vi "LoadCFG.vi"(8 "error in (no error)":errorcluster, 11 "object in":refnum<class "AIO-Configuration.lvclass">) -> (0 "error out":errorcluster, 2 "Success?":bool, 3 "object out":refnum<class "AIO-Configuration.lvclass">)   [LabVIEW 2021, in "DAQmx.lvlib" / "AIO-Configuration.lvclass"]
doc: "Loads Configuration"
uses:
  AIO-Configuration.lvclass
  C:/Users/averna/Documents/LV Gym DEMO/Factory Pattern/Channels/Dependencies/Channel.lvlibp/Channel/Configuration_class/Configuration.lvclass
  tdef/Data.ctl
  AIO-Configuration.lvclass/AIO-Configuration.ctl
  Dependencies/Channel.lvlibp/Channel/Configuration_class/properties/ReadConfigurationFile.vi
  <vilib>/Utility/config.llb/Read Key (String).vi
  <vilib>/Utility/config.llb/Read Key (Double).vi
  Dependencies/AIO-Channel.lvlibp/AIO-Configuration_class/AIO-Configuration.lvclass
  <vilib>/Utility/config.llb/NI_LVConfig.lvlib
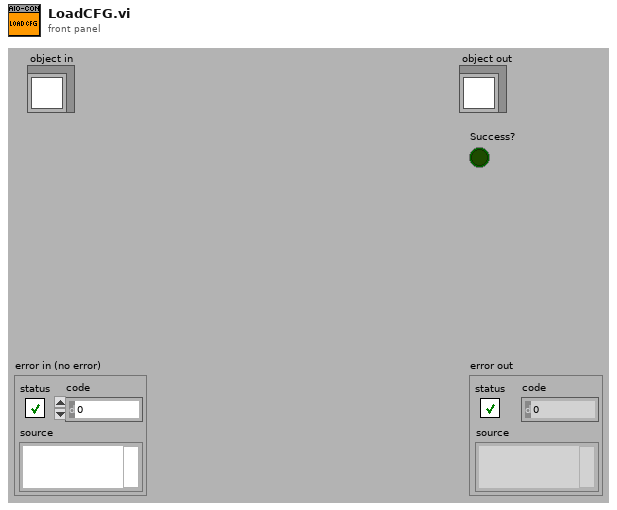
[diagram p1: front panel]
types:
  T1 = typedef "DAQmx.lvlib/AIO-Configuration.lvclass/Data.ctl" = cluster{"DAQ_Line":string, "maximum value":dbl, "minimum value":dbl, "input terminal configuration":i32, "custom scale name":string}
  T2 = typedef "NI_LVConfig.lvlib/Config Data RefNum.ctl" = refnum<k1>
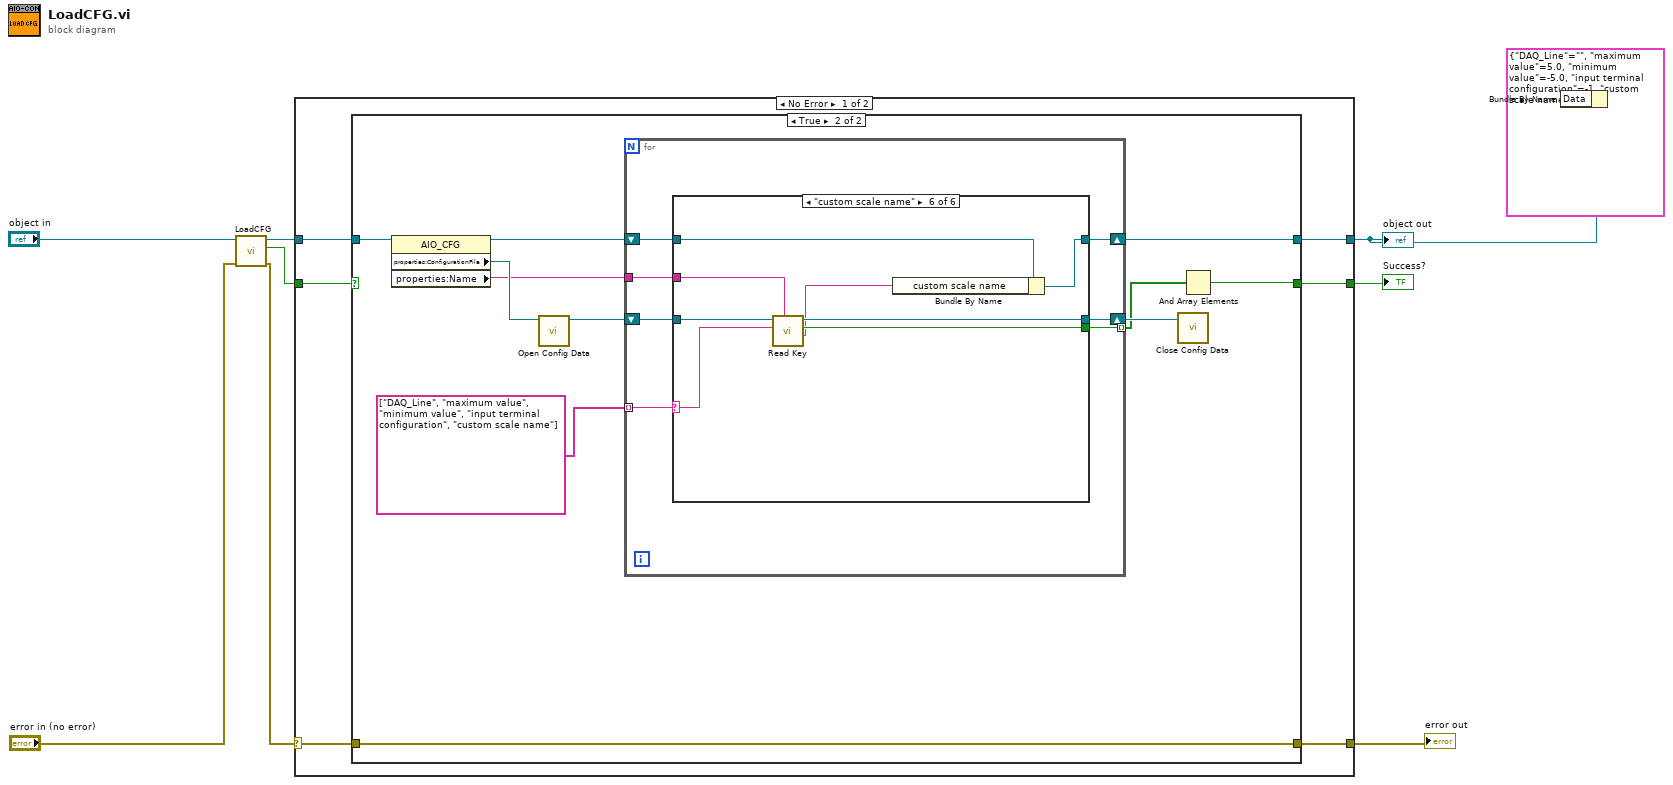
[diagram p0: block diagram]
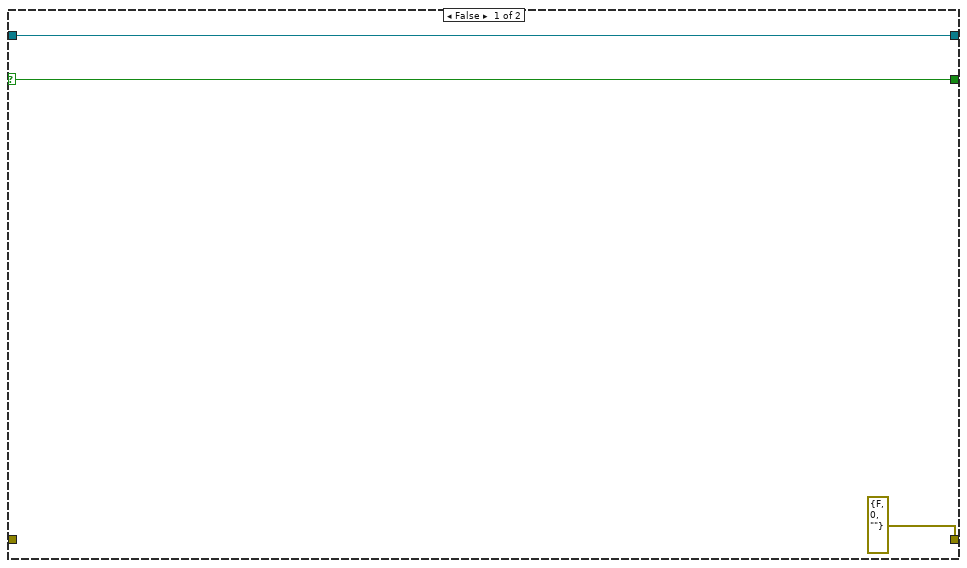
[diagram p2: hidden frame]
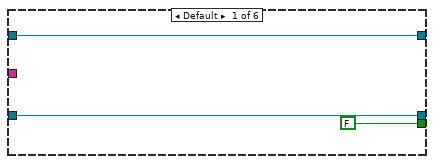
[diagram p3: hidden frame]
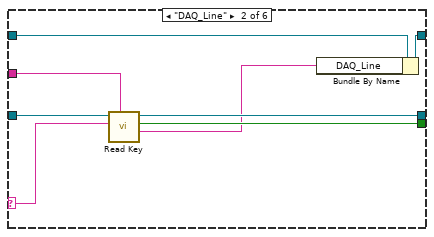
[diagram p4: hidden frame]
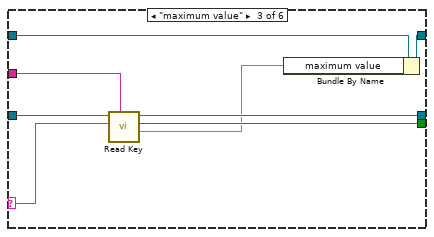
[diagram p5: hidden frame]
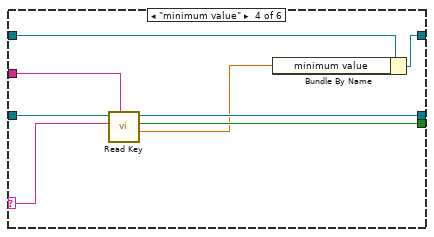
[diagram p6: hidden frame]
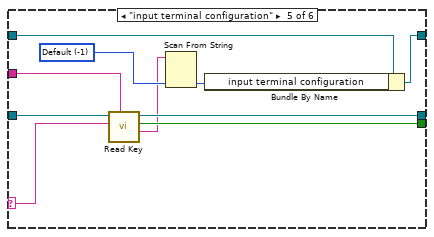
[diagram p7: hidden frame]
diagram:
  n1 = call-parent "LoadCFG.vi"("error in (no error)"="error in (no error)", "object in"="object in") -> ("error out"=w5:errorcluster, "Success?"=w6:bool, "object out"=w7:refnum<class "AIO-Configuration.lvclass">)  [unwired: 7 in]
  n2 = case shown="No Error" w5 {
    selector: w5 -> [w12 w84]
    tunnel: [w13 w84] -> w4
    tunnel: w7 -> [w14 w83]
    tunnel: [w10 w82] -> w3
    tunnel: w6 -> [w11 w82]
    tunnel: [w15 w83] -> w2
    frame No Error {
      n3 = case shown="True" w11 {
        selector: w11 -> [w17 _]
        tunnel: [w18 w25] -> w15
        tunnel: w14 -> [w18 w29]
        tunnel: [errorcluster {"status"=FALSE, "code"=0, "source"=""} ("error IO") w28] -> w13
        tunnel: w12 -> [_ w28]
        tunnel: [w17 w19] -> w10
        frame False {
        }
        frame True {
          n4 = property class="AIO_CFG"(reference=w29) -> (reference out=w24:refnum<class "AIO-Configuration.lvclass">, "properties:ConfigurationFile"=w27:path, "properties:Name"=w21:string)  [unwired: 1 in, 1 out]
          n5 = call <vilib>:"Open Config Data.vi"("configuration file path"=w27) -> ("refnum"=w26:T2)  [unwired: 8 in, 2 out]
          n6 = for {
            shift-right: [w32] -> w25
            shift-left: w24 -> [w31]
            shift-right: [w35] -> w23
            shift-left: w26 -> [w36]
            tunnel: string[] ["DAQ_Line", "maximum value", "minimum value", "input terminal configuration", "custom scale name"] -> [w34] mode=indexing
            tunnel: w21 -> [w33]
            tunnel: [w30] -> w20 mode=indexing
            n7 = case shown="\"custom scale name\"" w34 {
              selector: w34 -> [_ w45 w53 w61 w71 w79]
              tunnel: w36 -> [w38 w47 w55 w63 w73 w81]
              tunnel: [w38 w46 w54 w62 w72 w80] -> w35
              tunnel: w33 -> [_ w44 w52 w60 w70 w78]
              tunnel: [w39 w41 w49 w57 w67 w75] -> w32
              tunnel: w31 -> [w39 w43 w51 w59 w69 w77]
              tunnel: [FALSE ("found?") w42 w50 w58 w68 w76] -> w30
              frame Default {
              }
              frame "DAQ_Line" {
                n8 = call-poly <vilib>:"Read Key.vi"("section"=w44, "key"=w45, "refnum"=w47) -> ("value"=w40:string, "found?"=w42:bool, "refnum out"=w46:T2)  [unwired: 5 in, 1 out]
                n9 = Bundle By Name(cluster=w43, "DAQ_Line"=w40) -> (w41:refnum<class "AIO-Configuration.lvclass">)
              }
              frame "maximum value" {
                n10 = call-poly <vilib>:"Read Key.vi"("section"=w52, "key"=w53, "refnum"=w55) -> ("value"=w48:dbl, "found?"=w50:bool, "refnum out"=w54:T2)  [unwired: 5 in, 1 out]
                n11 = Bundle By Name(cluster=w51, "maximum value"=w48) -> (w49:refnum<class "AIO-Configuration.lvclass">)
              }
              frame "minimum value" {
                n12 = call-poly <vilib>:"Read Key.vi"("section"=w60, "key"=w61, "refnum"=w63) -> ("value"=w56:dbl, "found?"=w58:bool, "refnum out"=w62:T2)  [unwired: 5 in, 1 out]
                n13 = Bundle By Name(cluster=w59, "minimum value"=w56) -> (w57:refnum<class "AIO-Configuration.lvclass">)
              }
              frame "input terminal configuration" {
                w66 = -1 items=["Default"=-1, "RSE"=10083, "NRSE"=10078, "Differential"=10106, "Pseudodifferential"=12529] ("input terminal configuration")
                n14 = call-poly <vilib>:"Read Key.vi"("section"=w70, "key"=w71, "refnum"=w73) -> ("value"=w65:string, "found?"=w68:bool, "refnum out"=w72:T2)  [unwired: 5 in, 1 out]
                n15 = Scan From String(input string=w65, default 1=w66) -> (output 1=w64:i32)  [unwired: 3 in, 3 out]
                n16 = Bundle By Name(cluster=w69, "input terminal configuration"=w64) -> (w67:refnum<class "AIO-Configuration.lvclass">)
              }
              frame "custom scale name" {
                n17 = call-poly <vilib>:"Read Key.vi"("section"=w78, "key"=w79, "refnum"=w81) -> ("value"=w74:string, "found?"=w76:bool, "refnum out"=w80:T2)  [unwired: 5 in, 1 out]
                n18 = Bundle By Name(cluster=w77, "custom scale name"=w74) -> (w75:refnum<class "AIO-Configuration.lvclass">)
              }
            }
          }
          n19 = call <vilib>:"Close Config Data.vi"("refnum"=w23) -> ()  [unwired: 9 in, 2 out]
          n20 = And Array Elements(Boolean array=w20) -> (logical AND=w19:bool)
        }
      }
    }
    frame Error {
    }
  }
  "error out" <- w4
  "object out" <- w2
  "Success?" <- w3
  n21 = Bundle By Name(cluster=w2, "Data"=T1 {"DAQ_Line"="", "maximum value"=5.0, "minimum value"=-5.0, "input terminal configuration"=-1, "custom scale name"=""}) -> ()  [unwired: 1 out]
